vi "Main.vi"() -> ()   [LabVIEW 2021]
doc: "This Continuous Measurement sample project is based on the Queued Message Handler template.\n\nThe Event Handling Loop generates messages based on user interface actions.\n\nThe Message Handling Loop processes messages generated by the Event Handling Loop, or by other messages. There are also Acquisition and Logging message handling loop subVIs, and a chart updating loop."
uses:
  controls/Acquisition Status.ctl
  Settings/Settings.ctl
  Acquisition/Hardware Configuration.ctl
  Acquisition/Channel Settings.ctl
  Acquisition/IO Device.ctl
  Acquisition/Sensor Type.ctl
  Interval Timer/Repeat Interval.ctl
  Interval Timer/Interval Length.ctl
  Interval Timer/Interval Token.ctl
  Acquisition/IO Context.ctl
  Acquisition/IO API.ctl
  Logging/Logging Configuration.ctl
  Logging/Logging Mode.ctl
  Diagnostics/Diagnostics Configuration.ctl
  controls/Graph Settings.ctl
  controls/UI Data.ctl
  controls/UI State.ctl
  <vilib>/Utility/error.llb/DialogType.ctl
  support/Message Queue/Enqueue Message (Single).vi
  support/Message Queue/Enqueue Message (Array).vi
  <vilib>/Utility/error.llb/Error Cluster From Error Code.vi
  <vilib>/ErrorRing/Error Ring.xnode
  Acquisition/Acquisition.lvlib
  Logging/Logging.lvlib
  Settings/Settings.lvlib
  support/User Event - Stop/User Event - Stop.lvlib
  support/Message Queue/Message Queue.lvlib
  Settings/Settings Dialog.vi
  Diagnostics/Diagnostics.lvlib
  Interval Timer/Interval Timer.lvlib
panel:
  out "App Settings":T1
  out "Data":waveform(dbl)[](graph)
  in  "File Path":path
  out "Acquisition status":T15
  in  "Save Now":bool
  in  "Settings":bool
  in  "Start":bool
  in  "Stop":bool
  out "Status":string
  in  "Exit":bool
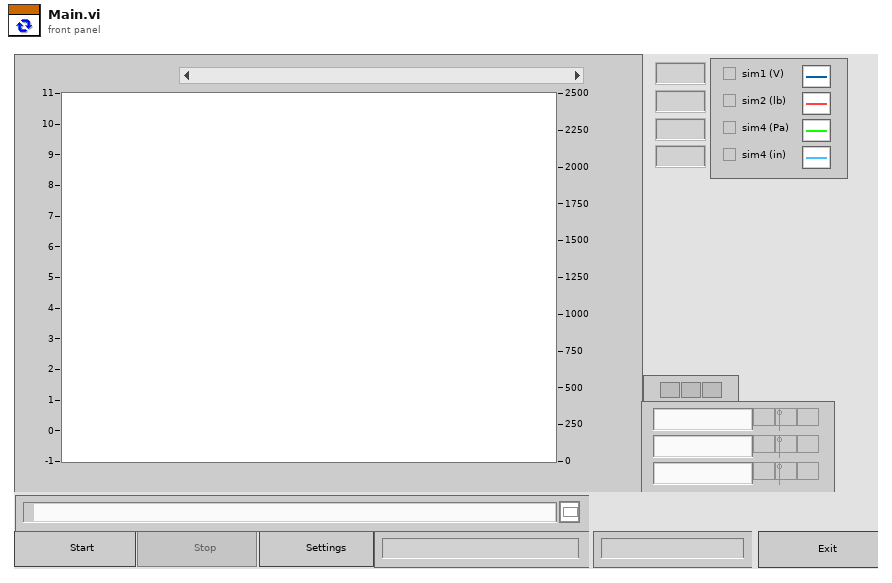
[diagram p1: front panel]
types:
  T1 = typedef "Settings.lvlib/Settings.ctl" = cluster{"IO":T2, "Log":T11, "Debug":T13, "Graph Settings":T14}
  T2 = typedef "Acquisition.lvlib/Hardware Configuration.ctl" = cluster{"Channel Settings":T3[], "Sensor Intervals":T6[], "Sensor Token":T8, "IO Context":T9}
  T3 = typedef "Acquisition.lvlib/Channel Settings.ctl" = cluster{"Name":string, "Terminal Information":cluster{"IO Device":T4, "Channel":i32, "Sensor Type":T5}, "Calibration Information":cluster{"Excitation Voltage":dbl, "Calibration Factor":dbl, "Zero Value":dbl, "Calibration Formula":string, "Units":string}}
  T4 = typedef "Acquisition.lvlib/IO Device.ctl" = enum16{"none", "9219", "9401"}
  T5 = typedef "Acquisition.lvlib/Sensor Type.ctl" = enum16{"Voltage", "Load", "Pressure", "Encoder"}
  T6 = typedef "Interval Timer.lvlib/Repeat Interval.ctl" = cluster{"Interval":T7, "Count":i32}
  T7 = typedef "Interval Timer.lvlib/Interval Length.ctl" = enum16{"Manual control", "1 second", "10 seconds", "30 seconds", "60 seconds", "600 seconds", "1200 seconds", "3600 seconds"}
  T8 = typedef "Interval Timer.lvlib/Interval Token.ctl" = cluster{"Next reading in ms":u32, "Interval Index":i32, "Interval Occurrence":i32}
  T9 = typedef "Acquisition.lvlib/IO Context.ctl" = cluster{"API":T10, "API Wire":variant}
  T10 = typedef "Acquisition.lvlib/IO API.ctl" = enum16{"Simulated", "DAQmx"}
  T11 = typedef "Logging.lvlib/Logging Configuration.ctl" = cluster{"Path":path, "Spreadsheet":refnum<file>, "Mode":T12}
  T12 = typedef "Logging.lvlib/Logging Mode.ctl" = enum16{"Overwrite", "Append", "Create New"}
  T13 = typedef "Diagnostics.lvlib/Diagnostics Configuration.ctl" = cluster{"Messages":refnum<file>}
  T14 = typedef "Graph Settings.ctl" = cluster{"Small Scale Max":dbl, "Large Scale Max":dbl, "Large Scale Threshold":dbl}
  T15 = typedef "Acquisition Status.ctl" = string
  T16 = typedef "UI State.ctl" = enum16{"Idle", "Acquiring and Logging", "Waiting for Exit", "Waiting for Exit (Acq Stopped)", "Waiting for Exit (Log Stopped)", "Waiting for Stop", "Waiting for Stop (Acq Stopped)", "Waiting for Stop (Log Stopped)"}
  T17 = typedef "UI Data.ctl" = cluster{"Start Ref":refnum<vi>, "Stop Ref":refnum<vi>, "Settings Ref":refnum<vi>, "Exit Ref":refnum<vi>, "Status Ref":refnum<vi>, "Data Ref":refnum<vi>, "Save Ref":refnum<vi>, "Path Ref":refnum<vi>}
  T18 = typedef "Acquisition.lvlib/Acquired Data.ctl" = cluster{"Waveform Array":waveform(dbl)[]}
  T19 = typedef "Message Queue.lvlib/All Message Queues.ctl" = cluster{"UI":refnum<queue>, "Acquisition":refnum<queue>, "Logging":refnum<queue>, "Diagnostic":refnum<queue>}
  T20 = typedef "Acquisition.lvlib/Host Resources.ctl" = cluster{"NI Software":T21[], "IO Devices":T22[]}
  T21 = typedef "Acquisition.lvlib/Host Software Package.ctl" = cluster{"ID":string, "Version":string}
  T22 = typedef "Acquisition.lvlib/Host IO Resource.ctl" = cluster{"Model Number":u32, "Alias":string, "Product Name":string, "Is Device":bool, "Is Chassis":bool, "Is Simulated":bool, "Slot":i32}
  T23 = typedef "DialogType.ctl" = u16
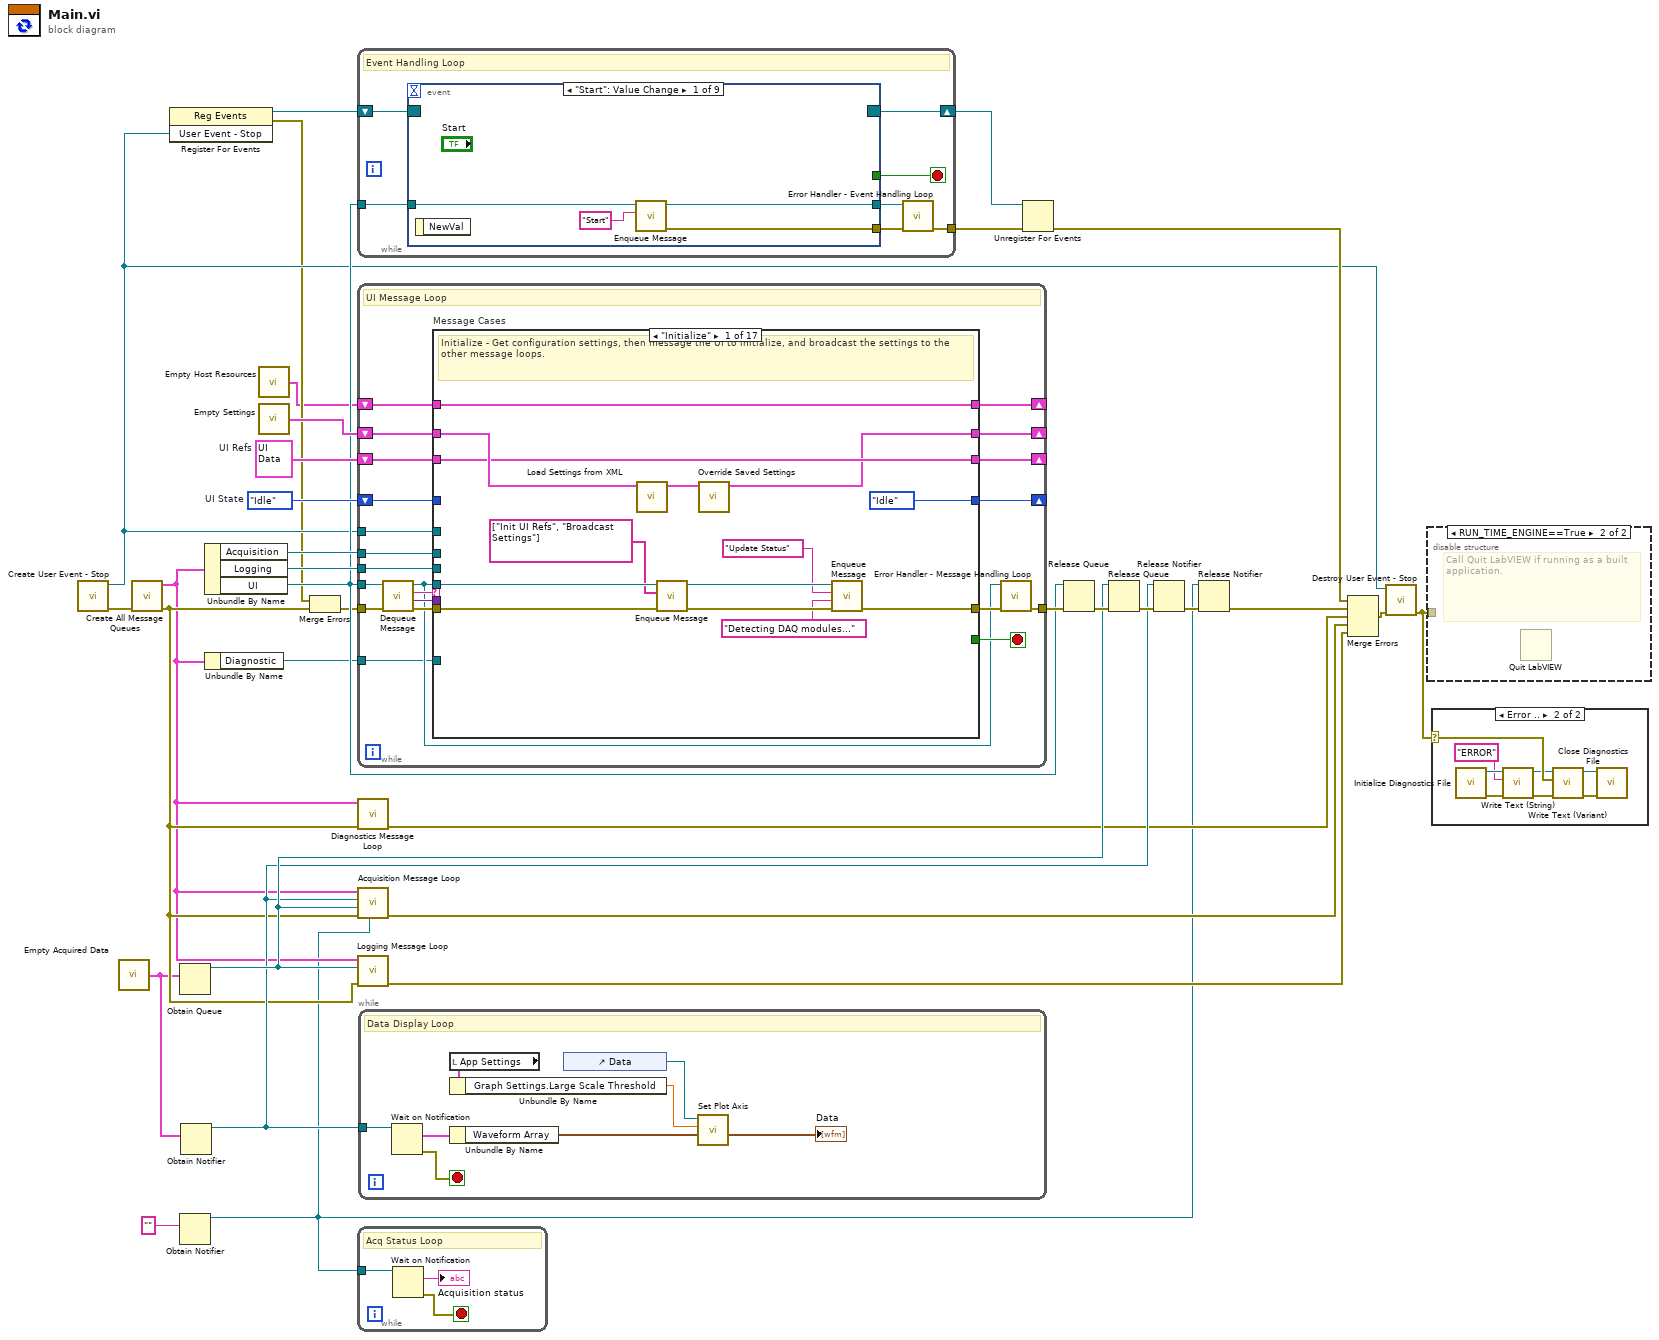
[diagram p0: block diagram]
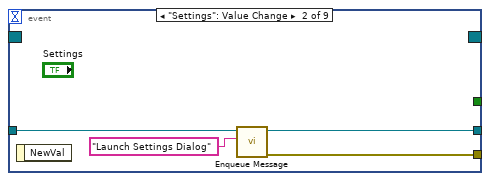
[diagram p4: hidden frame]
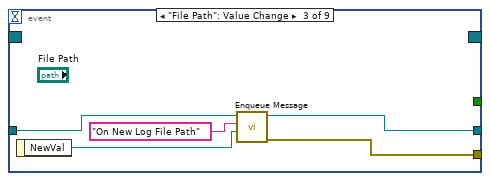
[diagram p5: hidden frame]
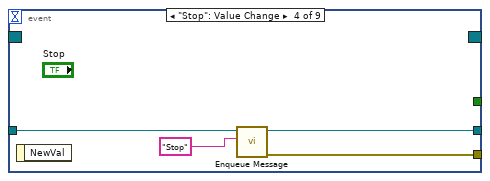
[diagram p6: hidden frame]
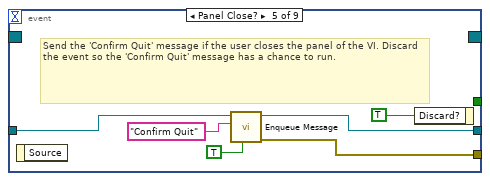
[diagram p7: hidden frame]
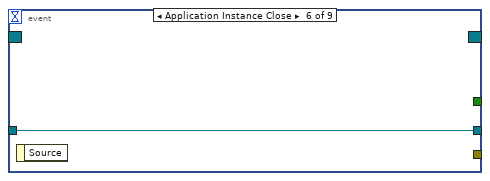
[diagram p8: hidden frame]
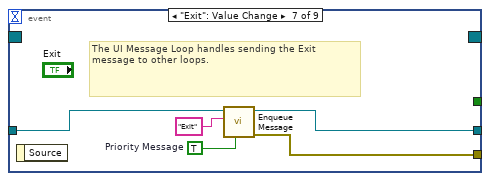
[diagram p9: hidden frame]
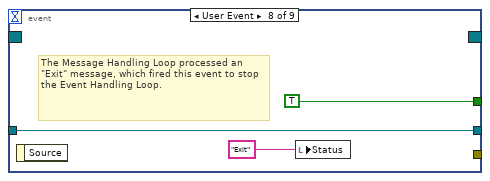
[diagram p10: hidden frame]
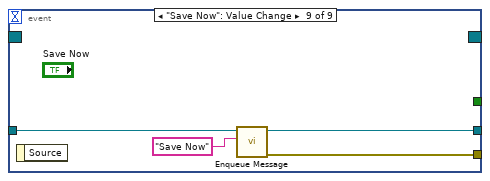
[diagram p11: hidden frame]
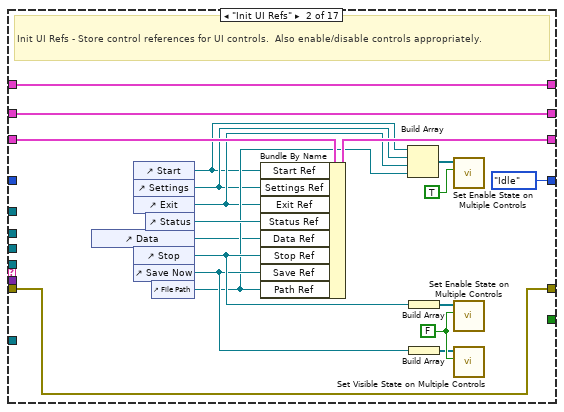
[diagram p12: hidden frame]
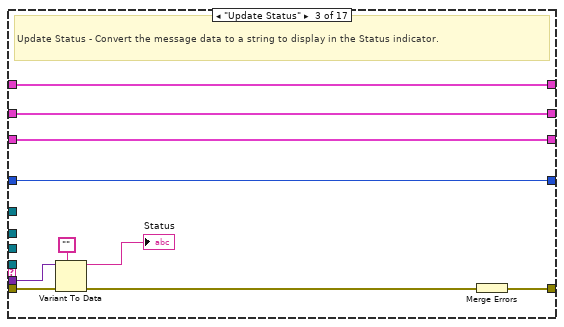
[diagram p13: hidden frame]
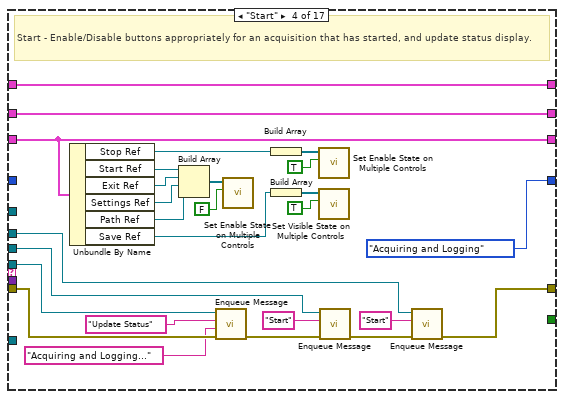
[diagram p14: hidden frame]
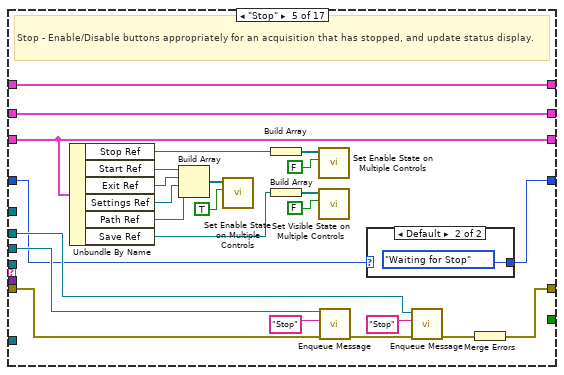
[diagram p15: hidden frame]
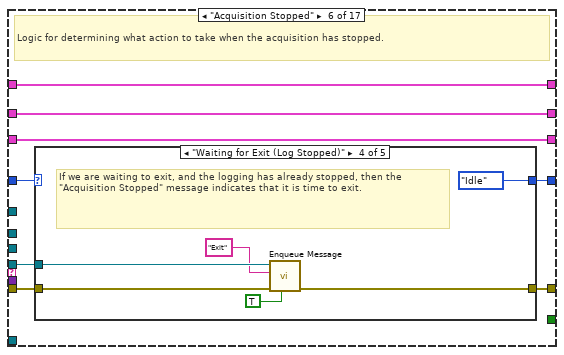
[diagram p17: hidden frame]
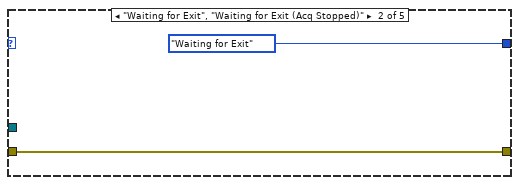
[diagram p19: hidden frame]
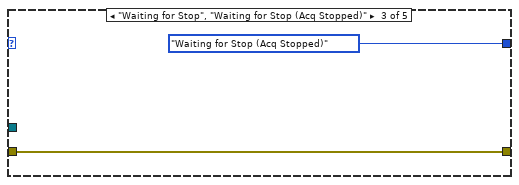
[diagram p20: hidden frame]
diagram:
  w22 = UI_State."Idle"  # UI State
  w25 = T17 {"Start Ref"=refnum, "Stop Ref"=refnum, "Settings Ref"=refnum, "Exit Ref"=refnum, "Status Ref"=refnum, "Data Ref"=refnum, "Save Ref"=refnum, "Path Ref"=refnum}  # UI Refs
  n1 = call "Create User Event - Stop.vi"() -> ("error out"=w30:errorcluster, "User Event - Stop"=w14:refnum<user-event>)  [unwired: 10 in]
  n2 = call "Empty Acquired Data.vi"() -> ("Empty Acquired Data"=w1:T18)
  n3 = call "Create All Message Queues.vi"("error in (no error)"=w30) -> ("error out"=w10:errorcluster, "Message Queues out"=w9:T19)  [unwired: 9 in]
  n4 = register-events(w14) -> (reference out=w15:refnum<event-registration>, error out=w12:errorcluster)  [unwired: 2 in]
  n5 = Obtain Queue(element data type=w1) -> (queue out=w17:refnum<queue>)  [unwired: 4 in, 2 out]
  n6 = Obtain Notifier(notification data type=T15 "") -> (notifier out=w3:refnum<notifier>)  [unwired: 3 in, 2 out]
  n7 = Obtain Notifier(notification data type=w1) -> (notifier out=w16:refnum<notifier>)  [unwired: 3 in, 2 out]
  n8 = Unbundle By Name(w9) -> ("Acquisition"=w24:refnum<queue>, "Logging"=w23:refnum<queue>, "UI"=w20:refnum<queue>)
  n9 = Unbundle By Name(w9) -> ("Diagnostic"=w11:refnum<queue>)
  n10 = call "Empty Host Resources.vi"() -> ("Host Resources"=w2:T20)
  n11 = call "Empty Settings.vi"() -> ("Settings"=w28:T1)
  n12 = Merge Errors(w12, w10) -> (w13:errorcluster)
  n13 = while {
    tunnel: w20 -> [w39]
    tunnel: [w36] -> w32
    shift-right: [w38] -> w26
    shift-left: w15 -> [w40]
    stop <- w37 stop-if-true
    # "Event Handling Loop"
    n14 = event shown="[0] \"Start\": Value Change" {
      selector: w40 -> [_ _ _ _ _ _ _ _ _]
      dyn-events: [_ _ _ _ _ _ _ _ _] -> w38
      timeout: _ -> [_ _ _ _ _ _ _ _ _]
      tunnel: [_ _ _ _ _ _ _ TRUE ("Discard?") _] -> w37
      tunnel: w39 -> [w44 w47 w52 w56 w61 w64 w66 w70 w76]
      tunnel: [w42 w45 w51 w55 w59 _ w69 _ w74] -> w35
      tunnel: [w41 w46 w49 w54 w60 w64 w65 w70 w75] -> w34
      event "Start": Value Change {
        n15 = event-data() -> ()  [unwired: 1 in, 1 out]
        n16 = call-poly "Enqueue Message.vi"("Message"="Start", "Message Queue"=w44) -> ("error out"=w42:errorcluster, "dup Message Queue"=w41:refnum<queue>)  [unwired: 8 in]
      }
      event "Settings": Value Change {
        n17 = event-data() -> ()  [unwired: 1 in, 1 out]
        n18 = call-poly "Enqueue Message.vi"("Message"="Launch Settings Dialog", "Message Queue"=w47) -> ("error out"=w45:errorcluster, "dup Message Queue"=w46:refnum<queue>)  [unwired: 8 in]
      }
      event "File Path": Value Change {
        n19 = event-data() -> ("NewVal"=w50:path)  [unwired: 1 in]
        n20 = call-poly "Enqueue Message.vi"("Message Data"=w50, "Message"="On New Log File Path", "Message Queue"=w52) -> ("error out"=w51:errorcluster, "dup Message Queue"=w49:refnum<queue>)  [unwired: 7 in]
      }
      event "Stop": Value Change {
        n21 = event-data() -> ()  [unwired: 1 in, 1 out]
        n22 = call-poly "Enqueue Message.vi"("Message"="Stop", "Message Queue"=w56) -> ("error out"=w55:errorcluster, "dup Message Queue"=w54:refnum<queue>)  [unwired: 8 in]
      }
      event Panel Close? {
        # "Send the 'Confirm Quit' message if the user closes the panel of the VI. Discard the event so the 'Confirm Quit' message has a chance to run."
        n23 = event-data() -> ()  [unwired: 1 in, 1 out]
        n24 = call-poly "Enqueue Message.vi"("Priority Message? (F)"=TRUE, "Message"="Confirm Quit", "Message Queue"=w61) -> ("error out"=w59:errorcluster, "dup Message Queue"=w60:refnum<queue>)  [unwired: 7 in]
        n25 = event-data("Discard?"=TRUE) -> ()  [unwired: 1 in, 1 out]
      }
      event Application Instance Close {
        n26 = event-data() -> ()  [unwired: 1 in, 1 out]
      }
      event "Exit": Value Change {
        w67 = TRUE  # Priority Message
        # "The UI Message Loop handles sending the Exit message to other loops."
        n27 = event-data() -> ()  [unwired: 1 in, 1 out]
        n28 = call-poly "Enqueue Message.vi"("Priority Message? (F)"=w67, "Message"="Exit", "Message Queue"=w66) -> ("error out"=w69:errorcluster, "dup Message Queue"=w65:refnum<queue>)  [unwired: 7 in]
      }
      event User Event {
        # "The Message Handling Loop processed an \"Exit\" message, which fired this event to stop the Event Handling Loop."
        n29 = event-data() -> ()  [unwired: 1 in, 1 out]
        n30 = local write "Status"("Exit" ("Exit String")) -> ()
      }
      event "Save Now": Value Change {
        n31 = event-data() -> ()  [unwired: 1 in, 1 out]
        n32 = call-poly "Enqueue Message.vi"("Message"="Save Now", "Message Queue"=w76) -> ("error out"=w74:errorcluster, "dup Message Queue"=w75:refnum<queue>)  [unwired: 8 in]
      }
    }
    n33 = call "Error Handler - Event Handling Loop.vi"("error in (no error)"=w35, "Message Queue"=w34) -> ("dup error in"=w36:errorcluster)  [unwired: 8 in, 1 out]
  }
  n34 = while {
    tunnel: w20 -> [w91]
    tunnel: w14 -> [w96]
    shift-right: [w90] -> _
    shift-left: w28 -> [w89]
    shift-right: [w87] -> _
    shift-left: w25 -> [w88]
    tunnel: w24 -> [w86]
    tunnel: w23 -> [w85]
    shift-right: [w80] -> _
    shift-left: w22 -> [w81]
    tunnel: w13 -> [w95]
    tunnel: [w84] -> w33
    tunnel: w11 -> [w79]
    shift-right: [w77] -> _
    shift-left: w2 -> [w78]
    stop <- w97 stop-if-true
    # "UI Message Loop"
    n35 = call "Dequeue Message.vi"("error in (no error)"=w95, "Message Queue"=w91) -> ("error out"=w94:errorcluster, "Message Data"=w92:variant, "Message"=w93:string, "dup Message Queue"=w82:refnum<queue>)  [unwired: 6 in]
    n36 = case "Message Cases" shown="\"Initialize\"" w93 {
      selector: w93 -> [_ _ _ _ _ _ _ _ _ _ _ _ _ _ _ _ w407]
      tunnel: w82 -> [w104 _ _ w167 _ w198 w224 _ w268 w286 w306 _ _ w359 w376 _ _]
      tunnel: w94 -> [w103 w118 w139 w166 w191 w199 w225 w258 w270 w292 w305 w343 w357 w371 w383 w399 _]
      tunnel: [w108 w118 w140 w150 w192 w196 w222 w250 w265 w294 w304 w350 w356 w373 w386 w404 w406] -> w83
      tunnel: [_ _ _ _ _ _ _ _ _ _ _ TRUE _ _ _ _ _] -> w97
      tunnel: w92 -> [_ _ w138 _ _ _ _ _ _ w295 _ w341 _ w370 w382 _ _]
      tunnel: w96 -> [_ _ _ _ _ _ _ _ _ _ _ w336 _ _ _ _ _]
      tunnel: [w98 w119 w134 w165 w190 w202 w228 w247 w262 w298 w309 w332 w355 w364 w378 w403 w410] -> w90
      tunnel: w89 -> [w111 w119 w134 w165 w190 w202 w228 w247 w271 w298 w309 w332 w355 w364 w380 w403 w410]
      tunnel: w88 -> [w105 w130 w133 w162 w189 w201 w227 w248 w266 w297 w308 w331 w354 w358 w385 w402 w409]
      tunnel: [w105 w128 w133 w162 w189 w201 w227 w248 w266 w297 w308 w331 w354 w358 w385 w402 w409] -> w87
      tunnel: w86 -> [_ _ _ w144 w176 _ _ w257 _ _ _ w349 _ _ _ w397 _]
      tunnel: w85 -> [_ _ _ w145 w179 _ _ w256 _ _ _ w348 _ _ _ _ _]
      tunnel: w81 -> [_ _ w132 _ w173 w200 w226 w255 w264 w293 w307 _ w353 w372 w384 w401 w408]
      tunnel: [UI_State."Idle" ("UI State") UI_State."Idle" ("UI State") w132 UI_State."Acquiring and Logging" ("UI State") w174 w197 w223 w255 w264 w293 w303 UI_State."Idle" ("UI State") w353 w372 w384 w401 w408] -> w80
      tunnel: w79 -> [_ _ _ _ _ _ _ w254 _ w280 _ w339 _ _ _ _ _]
      tunnel: w78 -> [w100 w117 w131 w143 w168 w195 w221 w249 w263 w291 w302 w333 w352 w368 w374 w396 w405]
      tunnel: [w100 w117 w131 w143 w168 w195 w221 w249 w263 w291 w302 w333 w352 w363 w374 w396 w405] -> w77
      frame "Initialize" {
        # "Initialize - Get configuration settings, then message the UI to initialize, and broadcast the settings to the other message loops."
        n37 = call "Load Settings from XML.vi"("Settings in"=w111) -> ("Settings out"=w99:T1)  [unwired: 9 in, 1 out]
        n38 = call-poly "Enqueue Message.vi"("error in (no error)"=w103, "Message Array"=string[] ["Init UI Refs", "Broadcast Settings"], "Message Queue"=w104) -> ("error out"=w110:errorcluster, "dup Message Queue"=w109:refnum<queue>)  [unwired: 7 in]
        n39 = call "Override Saved Settings.vi"("Settings in"=w99) -> ("Settings out"=w98:T1)  [unwired: 10 in]
        n40 = call-poly "Enqueue Message.vi"("error in (no error)"=w110, "Message Data"="Detecting DAQ modules..." ("Ready..."), "Message"="Update Status", "Message Queue"=w109) -> ("error out"=w108:errorcluster)  [unwired: 6 in, 1 out]
      }
      frame "Init UI Refs" {
        w122 = FALSE ("Enable?")
        # "Init UI Refs - Store control references for UI controls.  Also enable/disable controls appropriately."
        n41 = control-ref of="Data"() -> (w112:refnum<vi>)
        n42 = control-ref of="Start"() -> (w113:refnum<vi>)
        n43 = control-ref of="Settings"() -> (w114:refnum<vi>)
        n44 = control-ref of="Exit"() -> (w115:refnum<vi>)
        n45 = control-ref of="Stop"() -> (w123:refnum<vi>)
        n46 = control-ref of="Save Now"() -> (w120:refnum<vi>)
        n47 = control-ref of="Status"() -> (w129:refnum<vi>)
        n48 = control-ref of="File Path"() -> (w116:refnum<vi>)
        n49 = Bundle By Name(cluster=w130, "Start Ref"=w113, "Settings Ref"=w114, "Exit Ref"=w115, "Status Ref"=w129, "Data Ref"=w112, "Stop Ref"=w123, "Save Ref"=w120, "Path Ref"=w116) -> (w128:T17)
        n50 = Build Array(w113, w114, w115, w116) -> (w126:refnum<vi>[])
        n51 = Build Array(w123) -> (w125:refnum<vi>[])
        n52 = Build Array(w120) -> (w121:refnum<vi>[])
        n53 = call "Set Enable State on Multiple Controls.vi"("Enable?"=TRUE, "Controls"=w126) -> ()  [unwired: 9 in, 1 out]
        n54 = call "Set Enable State on Multiple Controls.vi"("Enable?"=w122, "Controls"=w125) -> ()  [unwired: 9 in, 1 out]
        n55 = call "Set Visible State on Multiple Controls.vi"("Visible?"=w122, "Controls"=w121) -> ()  [unwired: 10 in]
      }
      frame "Update Status" {
        # "Update Status - Convert the message data to a string to display in the Status indicator."
        n56 = Variant To Data(error in=w139, type="", Variant=w138) -> (data=→"Status":string, error out=w136:errorcluster)
        n57 = Merge Errors(w136) -> (w140:errorcluster)
      }
      frame "Start" {
        # "Start - Enable/Disable buttons appropriately for an acquisition that has started, and update status display."
        n58 = Unbundle By Name(w162) -> ("Stop Ref"=w157:refnum<vi>, "Start Ref"=w156:refnum<vi>, "Exit Ref"=w155:refnum<vi>, "Settings Ref"=w154:refnum<vi>, "Path Ref"=w142:refnum<vi>, "Save Ref"=w141:refnum<vi>)
        n59 = Build Array(w156, w155, w154, w142) -> (w160:refnum<vi>[])
        n60 = call-poly "Enqueue Message.vi"("error in (no error)"=w166, "Message Data"="Acquiring and Logging..." ("Acquiring and Logging..."), "Message"="Update Status", "Message Queue"=w167) -> ("error out"=w153:errorcluster)  [unwired: 6 in, 1 out]
        n61 = call "Set Enable State on Multiple Controls.vi"("Enable?"=FALSE, "Controls"=w160) -> ()  [unwired: 9 in, 1 out]
        n62 = Build Array(w157) -> (w159:refnum<vi>[])
        n63 = Build Array(w141) -> (w147:refnum<vi>[])
        n64 = call "Set Enable State on Multiple Controls.vi"("Enable?"=TRUE, "Controls"=w159) -> ()  [unwired: 9 in, 1 out]
        n65 = call "Set Visible State on Multiple Controls.vi"("Visible?"=TRUE ("Visble?"), "Controls"=w147) -> ()  [unwired: 10 in]
        n66 = call-poly "Enqueue Message.vi"("error in (no error)"=w153, "Message"="Start", "Message Queue"=w145) -> ("error out"=w151:errorcluster)  [unwired: 7 in, 1 out]
        n67 = call-poly "Enqueue Message.vi"("error in (no error)"=w151, "Message"="Start", "Message Queue"=w144) -> ("error out"=w150:errorcluster)  [unwired: 7 in, 1 out]
      }
      frame "Stop" {
        # "Stop - Enable/Disable buttons appropriately for an acquisition that has stopped, and update status display."
        n68 = Unbundle By Name(w189) -> ("Stop Ref"=w184:refnum<vi>, "Start Ref"=w169:refnum<vi>, "Exit Ref"=w183:refnum<vi>, "Settings Ref"=w182:refnum<vi>, "Path Ref"=w181:refnum<vi>, "Save Ref"=w170:refnum<vi>)
        n69 = Build Array(w169, w183, w182, w181) -> (w187:refnum<vi>[])
        n70 = call "Set Enable State on Multiple Controls.vi"("Enable?"=TRUE, "Controls"=w187) -> ()  [unwired: 9 in, 1 out]
        n71 = Build Array(w184) -> (w186:refnum<vi>[])
        n72 = Build Array(w170) -> (w172:refnum<vi>[])
        n73 = call "Set Enable State on Multiple Controls.vi"("Enable?"=FALSE, "Controls"=w186) -> ()  [unwired: 9 in, 1 out]
        n74 = call "Set Visible State on Multiple Controls.vi"("Visible?"=FALSE ("Enable?"), "Controls"=w172) -> ()  [unwired: 10 in]
        n75 = call-poly "Enqueue Message.vi"("error in (no error)"=w191, "Message"="Stop", "Message Queue"=w179) -> ("error out"=w178:errorcluster)  [unwired: 7 in, 1 out]
        n76 = case shown="Default" w173 {
          selector: w173 -> [w193 _]
          tunnel: [w193 UI_State."Waiting for Stop" ("UI State")] -> w174
          frame "Waiting for Exit" {
          }
          frame Default {
          }
        }
        n77 = call-poly "Enqueue Message.vi"("error in (no error)"=w178, "Message"="Stop", "Message Queue"=w176) -> ("error out"=w177:errorcluster)  [unwired: 7 in, 1 out]
        n78 = Merge Errors(w177) -> (w192:errorcluster)
      }
      frame "Acquisition Stopped" {
        # "Logic for determining what action to take when the acquisition has stopped."
        n79 = case shown="\"Waiting for Exit (Log Stopped)\"" w200 {
          selector: w200 -> [w204 _ _ _ _]
          tunnel: w199 -> [w203 w206 w208 w214 w220]
          tunnel: w198 -> [_ _ _ w212 w217]
          tunnel: [w204 UI_State."Waiting for Exit" ("UI State") UI_State."Waiting for Stop (Acq Stopped)" ("UI State") UI_State."Idle" ("UI State") UI_State."Idle" ("UI State")] -> w197
          tunnel: [w203 w206 w208 w213 w218] -> w196
          frame Default {
          }
          frame "Waiting for Exit", "Waiting for Exit (Acq Stopped)" {
          }
          frame "Waiting for Stop", "Waiting for Stop (Acq Stopped)" {
          }
          frame "Waiting for Exit (Log Stopped)" {
            # "If we are waiting to exit, and the logging has already stopped, then the \"Acquisition Stopped\" message indicates that it is time to exit."
            n80 = call-poly "Enqueue Message.vi"("Priority Message? (F)"=TRUE, "error in (no error)"=w214, "Message"="Exit", "Message Queue"=w212) -> ("error out"=w213:errorcluster)  [unwired: 6 in, 1 out]
          }
          frame "Waiting for Stop (Log Stopped)" {
            # "If we are waiting to stop, and the logging has already stopped, then the \"Acquisition Stopped\" message indicates that it is time to stop."
            n81 = call-poly "Enqueue Message.vi"("error in (no error)"=w220, "Message Data"="Ready..." ("Ready..."), "Message"="Update Status", "Message Queue"=w217) -> ("error out"=w218:errorcluster)  [unwired: 6 in, 1 out]
          }
        }
      }
      frame "Logging Stopped" {
        # "Logic for determining what action to take when the logging has stopped."
        n82 = case shown="\"Waiting for Stop (Acq Stopped)\"" w226 {
          selector: w226 -> [w230 _ _ _ _]
          tunnel: w225 -> [w229 w232 w234 w240 w243]
          tunnel: w224 -> [_ _ _ w238 w242]
          tunnel: [w230 UI_State."Waiting for Exit (Log Stopped)" ("UI State") UI_State."Waiting for Stop (Log Stopped)" ("UI State") UI_State."Idle" ("UI State") UI_State."Idle" ("UI State")] -> w223
          tunnel: [w229 w232 w234 w239 w241] -> w222
          frame Default {
          }
          frame "Waiting for Exit", "Waiting for Exit (Log Stopped)" {
          }
          frame "Waiting for Stop", "Waiting for Stop (Log Stopped)" {
          }
          frame "Waiting for Exit (Acq Stopped)" {
            # "If we are waiting to exit, and the acquisition has already stopped, then the \"Logging Stopped\" message indicates that it is time to exit."
            n83 = call-poly "Enqueue Message.vi"("Priority Message? (F)"=TRUE, "error in (no error)"=w240, "Message"="Exit", "Message Queue"=w238) -> ("error out"=w239:errorcluster)  [unwired: 6 in, 1 out]
          }
          frame "Waiting for Stop (Acq Stopped)" {
            # "If we are waiting to stop, and the acquisition has already stopped, then the \"Logging Stopped\" message indicates that it is time to stop."
            n84 = call-poly "Enqueue Message.vi"("error in (no error)"=w243, "Message Data"="Ready..." ("Ready..."), "Message"="Update Status", "Message Queue"=w242) -> ("error out"=w241:errorcluster)  [unwired: 6 in, 1 out]
          }
        }
      }
      frame "Broadcast settings" {
        w252 = "Update Settings" ("Message")
        # "Broadcast settings - Send the 'Update Settings' message to the Logging and Acquisition message loops."
        n85 = Unbundle By Name(w247) -> ("IO"=w260:T2)
        n86 = call-poly "Enqueue Message.vi"("Message Data"=w260, "Message"=w252, "Message Queue"=w257) -> ("error out"=w261:errorcluster)  [unwired: 7 in, 1 out]
        n87 = call-poly "Enqueue Message.vi"("error in (no error)"=w261, "Message Data"=w247, "Message"=w252, "Message Queue"=w256) -> ("error out"=w259:errorcluster)  [unwired: 6 in, 1 out]
        n88 = call-poly "Enqueue Message.vi"("Message Data"=w247, "Message"=w252, "Message Queue"=w254) -> ("error out"=w253:errorcluster)  [unwired: 7 in, 1 out]
        n89 = Merge Errors(w259, w258, w253) -> (w251:errorcluster)
        n90 = call "Apply Settings.vi"("Host"=w249, "error in (no error)"=w251, "Measurement UI Controls"=w248, "Settings"=w247) -> ("error out"=w250:errorcluster)  [unwired: 6 in, 1 out]
        "App Settings" <- w247
      }
      frame "Launch Settings Dialog" {
        # "Launch Settings Dialog - Launch the Settings Dialog when the user clicks the 'Settings' button."
        n91 = call-by-ref "?"("Host"=w263, "error in (no error)"=w270, "Settings in"=w271) -> ("error out"=w267:errorcluster, "Cancelled?"=w269:bool, "Settings out"=w262:T1)  [unwired: 8 in, 2 out]
        n92 = case shown="False" w269 {
          tunnel: w268 -> [w276 _]
          tunnel: w267 -> [w275 w277]
          tunnel: [w274 w277] -> w265
          tunnel: w262 -> [w272 _]
          frame False {
            n93 = call "Save Settings to XML.vi"("Settings"=w272) -> ()  [unwired: 10 in, 1 out]
            n94 = call-poly "Enqueue Message.vi"("error in (no error)"=w275, "Message"="Broadcast Settings", "Message Queue"=w276) -> ("error out"=w274:errorcluster)  [unwired: 7 in, 1 out]
          }
          frame True {
          }
        }
      }
      frame "Error" {
        w290 = T23 0 items=["no dialog", "OK message", "continue or stop message", "OK message + warnings", "continue/stop + warnings"] ("type of dialog (OK msg:1)")
        # "Error - Display an error dialog. This message is sent by the \"Error Handler\" VIs at the end of other loops in this application."
        n95 = Variant To Data(error in=w292, type=errorcluster {"status"=FALSE, "code"=0, "source"=""} ("error constant"), Variant=w295) -> (data=w288:errorcluster, error out=w289:errorcluster)
        n96 = call <vilib>:"Simple Error Handler.vi"("type of dialog (OK msg:1)"=w290, "error in (no error)"=w288) -> ("source out"=w282:string, "message"=w281:string)  [unwired: 3 in, 3 out]
        n97 = Format Into String(format string="Unhandled runtime error\n\n%s%s", w282, w281) -> (resulting string=w278:string)  [unwired: 2 in, 1 out]
        n98 = call-poly "Enqueue Message.vi"("Message Data"=w278, "Message"="Trace", "Message Queue"=w280) -> ()  [unwired: 7 in, 2 out]
        n99 = Two Button Dialog(message=w278, 1:"Exit" ("F button name (\"Cancel\")"), 2:"Continue" ("T button name (\"OK\")")) -> (T button?=w287:bool)
        n100 = case shown="False" w287 {
          tunnel: w286 -> [w301 _]
          frame False {
            n101 = call-poly "Enqueue Message.vi"("Priority Message? (F)"=TRUE, "Message"="Exit", "Message Queue"=w301) -> ()  [unwired: 7 in, 2 out]
          }
          frame True {
          }
        }
        n102 = Merge Errors(w289) -> (w294:errorcluster)
      }
      frame "Confirm Quit" {
        # "Confirm Quit - Message that can confirm whether or not the user wants to exit the application."
        n103 = case shown="\"Acquiring and Logging\"" w307 {
          tunnel: w306 -> [w315 w319]
          tunnel: w305 -> [w314 w318]
          tunnel: [w313 w317] -> w304
          tunnel: [UI_State."Idle" ("UI State") w316] -> w303
          frame Default {
            # "If 'Confirm Quit' comes in while the system is idle, there is no need for a confirmation message."
            n104 = call-poly "Enqueue Message.vi"("Priority Message? (F)"=TRUE, "error in (no error)"=w314, "Message"="Exit", "Message Queue"=w315) -> ("error out"=w313:errorcluster)  [unwired: 6 in, 1 out]
          }
          frame "Acquiring and Logging" {
            n105 = Two Button Dialog(message="Are you sure you want to quit while the acquisition is running?" ("Confirm Quit Message"), 1:"No" ("No"), 2:"Yes" ("Yes")) -> (T button?=w320:bool)
            n106 = case shown="True" w320 {
              tunnel: w319 -> [_ w329]
              tunnel: w318 -> [w325 w330]
              tunnel: [w325 w328] -> w317
              tunnel: [UI_State."Acquiring and Logging" ("UI State") UI_State."Waiting for Exit" ("UI State")] -> w316
              frame False {
                # "User did not want to quit."
              }
              frame True {
                n107 = call-poly "Enqueue Message.vi"("error in (no error)"=w330, "Message"="Stop", "Message Queue"=w329) -> ("error out"=w328:errorcluster)  [unwired: 7 in, 1 out]
              }
            }
          }
        }
      }
      frame "Exit" {
        w345 = TRUE ("Priority Message? (F)")
        w338 = "Exit" ("Message")
        # "Popup an error dialog if 'Exit' was called as a result of an error."
        # "Stop the VI"
        # "Exit - Send Exit messages to the Acquisition and Logging loops, and fire the user event to stop the Event Handling Loop."
        n108 = Variant To Data(type=errorcluster {"status"=FALSE, "code"=0, "source"=""} ("error constant"), Variant=w341) -> (data=w340:errorcluster)  [unwired: 1 in, 1 out]
        n109 = call <vilib>:"Simple Error Handler.vi"("error in (no error)"=w340) -> ()  [unwired: 4 in, 5 out]
        n110 = call-poly "Enqueue Message.vi"("Priority Message? (F)"=w345, "error in (no error)"=w343, "Message"=w338, "Message Queue"=w349) -> ("error out"=w346:errorcluster)  [unwired: 6 in, 1 out]
        n111 = call-poly "Enqueue Message.vi"("Message"=w338, "Message Queue"=w339) -> ("error out"=w337:errorcluster)  [unwired: 8 in, 1 out]
        n112 = call-poly "Enqueue Message.vi"("Priority Message? (F)"=w345, "error in (no error)"=w346, "Message"=w338, "Message Queue"=w348) -> ("error out"=w344:errorcluster)  [unwired: 6 in, 1 out]
        n113 = Merge Errors(w344, w337) -> (w335:errorcluster)
        n114 = call "Reset UI Colors.vi"("Host"=w333, "error in (no error)"=w335, "Measurement UI Controls"=w331, "Settings"=w332) -> ("error out"=w334:errorcluster)  [unwired: 6 in, 1 out]
        n115 = call "Invoke User Event - Stop.vi"("error in (no error)"=w334, "User Event - Stop"=w336) -> ("error out"=w350:errorcluster)  [unwired: 9 in]
      }
      frame "---Copy This Frame---" {
        # "Duplicate this frame when creating new messages.  Change this comment in the duplicated frame to describe this message."
        n116 = Merge Errors(w357) -> (w356:errorcluster)
      }
      frame "On IO Discovery Complete" {
        # "When the Acquisition Loop finishes handling the Initialize message, it sends this message back to update the program with the resources like software, drivers, hardware on the system."
        n117 = call "Empty Host Resources.vi"() -> ("Host Resources"=w369:T20)
        n118 = Variant To Data(error in=w371, type=w369, Variant=w370) -> (data=w367:T20, error out=w362:errorcluster)
        n119 = Select(t=w368, s=w362, f=w367) -> (s? t:f=w363:T20)
        n120 = call "Update Settings button colors.vi"("Host in"=w363, "error in (no error)"=w362, "Measurement UI Controls"=w358, "Settings in"=w364) -> ("error out"=w361:errorcluster)  [unwired: 6 in, 1 out]
        n121 = call-poly "Enqueue Message.vi"("error in (no error)"=w361, "Message Data"="Ready..." ("Ready..."), "Message"="Update Status", "Message Queue"=w359) -> ("error out"=w360:errorcluster)  [unwired: 6 in, 1 out]
        n122 = Merge Errors(w360) -> (w373:errorcluster)
      }
      frame "On New Log File Path" {
        # "Update the log file in settings and broadcast to other loops."
        n123 = Variant To Data(error in=w383, type=path "", Variant=w382) -> (data=w379:path, error out=w375:errorcluster)
        n124 = case shown="No Error" w375 {
          selector: w375 -> [w387 w395]
          tunnel: w380 -> [w393 w394]
          tunnel: w379 -> [w392 _]
          tunnel: [w391 w394] -> w378
          tunnel: [w389 w395] -> w377
          tunnel: w376 -> [w388 _]
          frame No Error {
            n125 = Bundle By Name(cluster=w393, "Log.Path"=w392) -> (w391:T1)
            n126 = call-poly "Enqueue Message.vi"("error in (no error)"=w387, "Message"="Broadcast Settings", "Message Queue"=w388) -> ("error out"=w389:errorcluster)  [unwired: 7 in, 1 out]
          }
          frame Error {
          }
        }
        n127 = Merge Errors(w377) -> (w386:errorcluster)
      }
      frame "Save Now" {
        # "Take a measurement on-demand."
        n128 = call-poly "Enqueue Message.vi"("error in (no error)"=w399, "Message"="Save Now", "Message Queue"=w397) -> ("error out"=w398:errorcluster)  [unwired: 7 in, 1 out]
        n129 = Merge Errors(w398) -> (w404:errorcluster)
      }
      frame Default {
        # "'Default' case only runs if there is a message that isn't defined in any of the other cases.  Output a programming error."
        n130 = xnode "Error Ring"("parameter 0"=w407) -> ("error out"=w406:errorcluster)
      }
    }
    n131 = call "Error Handler - Message Handling Loop.vi"("error in (no error)"=w83, "Message Queue"=w82) -> ("dup error in"=w84:errorcluster)  [unwired: 8 in, 1 out]
  }
  n132 = call "Diagnostics Message Loop.vi"("error in (no error)"=w10, "Message Queues"=w9) -> ("error out"=w8:errorcluster)  [unwired: 9 in]
  n133 = call "Acquisition Message Loop.vi"("Acquisition Status Notifier"=w3, "error in (no error)"=w10, "Data Queue"=w17, "Data Notifier"=w16, "Message Queues"=w9) -> ("error out"=w31:errorcluster)  [unwired: 6 in]
  n134 = call "Logging Message Loop.vi"("error in (no error)"=w10, "Data Queue"=w17, "Message Queues"=w9) -> ("error out"=w29:errorcluster)  [unwired: 8 in]
  n135 = while {
    tunnel: w3 -> [w418]
    stop <- w420 stop-if-true
    # "Acq Status Loop"
    n136 = Wait on Notification(notifier=w418) -> (notification=→"Acquisition status":T15, error out=w420:errorcluster)  [unwired: 3 in, 2 out]
  }
  n137 = while "Data Display Loop" {
    tunnel: w16 -> [w428]
    stop <- w427 stop-if-true
    # "Data Display Loop"
    n138 = Wait on Notification(notifier=w428) -> (notification=w426:T18, error out=w427:errorcluster)  [unwired: 3 in, 2 out]
    n139 = local read "App Settings"() -> (w422:T1)
    n140 = Unbundle By Name(w422) -> ("Graph Settings.Large Scale Threshold"=w421:dbl)
    n141 = Unbundle By Name(w426) -> ("Waveform Array"=w424:waveform(dbl)[])
    n142 = control-ref of="Data"() -> (w425:refnum<vi>)
    n143 = call "Set Plot Axis.vi"("Waveform Array"=w424, "Large Scale threshold"=w421, "Waveform Chart ref"=w425) -> ("Waveform Array out"=→"Data":waveform(dbl)[])  [unwired: 7 in, 1 out]
  }
  n144 = Unregister For Events(event registration refnum=w26, error in=w32) -> (error out=w27:errorcluster)
  n145 = Release Queue(queue=w20, error in (no error)=w33) -> (error out=w19:errorcluster)  [unwired: 1 in, 2 out]
  n146 = Release Queue(queue=w17, error in (no error)=w19) -> (error out=w18:errorcluster)  [unwired: 1 in, 2 out]
  n147 = Release Notifier(notifier=w16, error in (no error)=w18) -> (error out=w5:errorcluster)  [unwired: 1 in, 2 out]
  n148 = Release Notifier(notifier=w3, error in (no error)=w5) -> (error out=w4:errorcluster)  [unwired: 1 in, 2 out]
  n149 = Merge Errors(w27, w4, w8, w31, w29) -> (w21:errorcluster)
  n150 = call "Destroy User Event - Stop.vi"("error in (no error)"=w21, "User Event - Stop"=w14) -> ("error out"=w7:errorcluster)  [unwired: 9 in]
  n151 = disable-structure shown="RUN_TIME_ENGINE==True" {
    disable-tunnel: w7 -> [_ _]
    frame condition #0 (active) {
    }
    frame condition #1 {
      # "Call Quit LabVIEW if running as a built application."
      n152 = Quit LabVIEW() -> ()  [unwired: 1 in]
    }
  }
  n153 = case shown="Error .." w7 {
    selector: w7 -> [_ w434]
    frame No Error {
    }
    frame Error {
      n154 = call "Initialize Diagnostics File.vi"() -> ("error out"=w433:errorcluster, "diagnostics file"=w430:refnum<file>)  [unwired: 10 in]
      n155 = call "Write Text (String).vi"("error in"=w433, "String"="ERROR", "file in"=w430) -> ("error out"=w432:errorcluster, "file out"=w431:refnum<file>)  [unwired: 7 in]
      n156 = call "Write Text (Variant).vi"("error in"=w432, "Anything"=w434, "file in"=w431) -> ("error out"=w436:errorcluster, "file out"=w435:refnum<file>)  [unwired: 7 in]
      n157 = call "Close Diagnostics File.vi"("error in"=w436, "diagnostics file"=w435) -> ()  [unwired: 8 in, 2 out]
    }
  }
